vi "JSON RPC Engine.vi"(8 "error in (no error)":errorcluster, 10 "methods directory":path) -> (0 "error out":errorcluster)   [LabVIEW 2017, in "JSONRPC Server.lvclass"]
doc: "Use this as a starting point for the RPC Server processing loop in your application"
uses:
  JSONRPC Server.lvclass
  Request/Request.lvclass/Request.ctl
  Request/request.Read method.vi
  Request/request.Read params.vi
  params/params.To JSON Tree.vi
  Add Response (Method Not Found from Request).vi
  Add Response (Result from Request).vi
  Add Response (Server Error from Request).vi
  Add Response (Internal Error from Request).vi
  Method Loader/Method Loader.lvclass
  Request/Request.lvclass
  <vilib>/National Instruments/Variant JSON API/Variant JSON API.lvlib
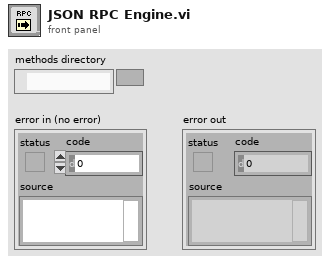
[diagram p1: front panel]
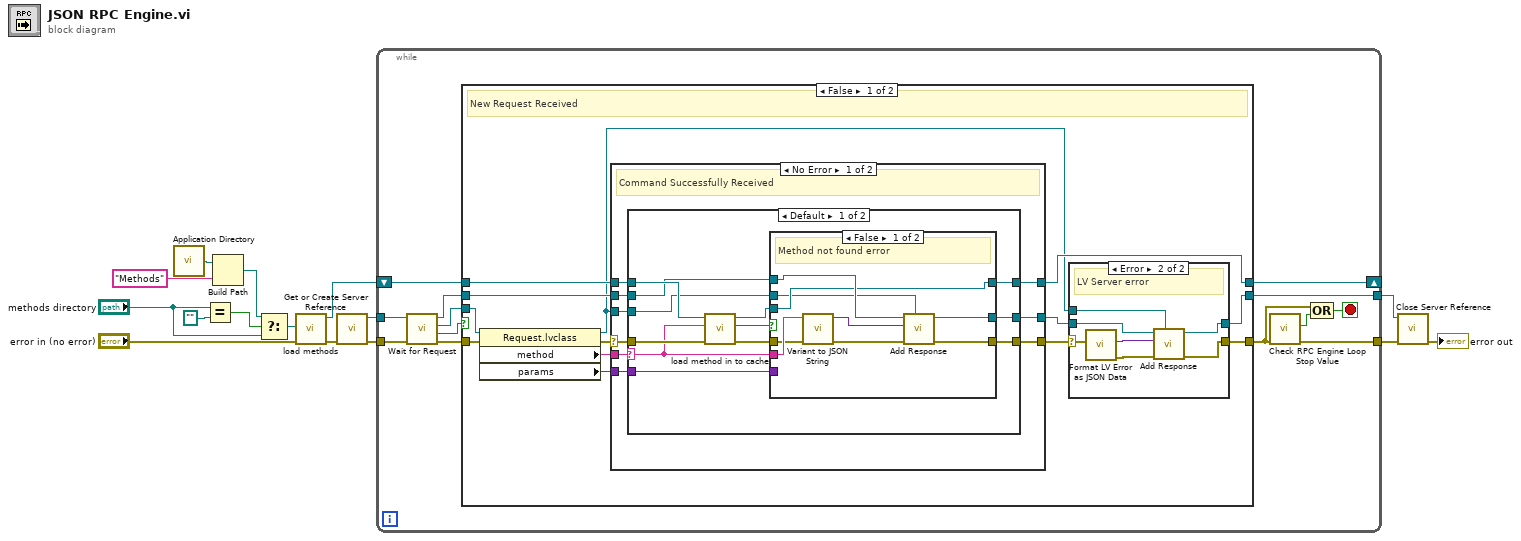
[diagram p0: block diagram]
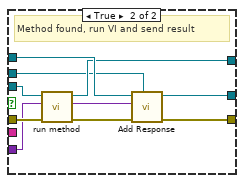
[diagram p3: hidden frame]
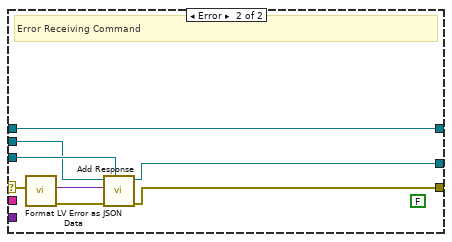
[diagram p5: hidden frame]
diagram:
  n1 = call <vilib>:"Application Directory.vi"() -> ("Application Directory"=w11:path)
  n2 = Equal?(x="methods directory", y=path "") -> (x = y?=w4:bool)
  n3 = Build Path(base path=w11, name or relative path="Methods") -> (appended path=w3:path)
  n4 = Select(t=w3, s=w4, f="methods directory") -> (s? t:f=w1:path)
  n5 = call "load methods.vi"("error in (no error)"="error in (no error)", "Folder Path"=w1) -> ("error out"=w9:errorcluster, "Method Manager out"=w8:refnum<class "Method Loader.lvclass">)  [unwired: 8 in]
  n6 = call "Get or Create Server Reference.vi"("error in (no error)"=w9) -> ("error out"=w14:errorcluster, "Server Out"=w15:refnum<class "JSONRPC Server.lvclass">)  [unwired: 9 in]
  n7 = while {
    tunnel: w15 -> [w28]
    tunnel: w14 -> [w24]
    tunnel: [w17] -> w12
    tunnel: [w22] -> w13
    shift-right: [w19] -> _
    shift-left: w8 -> [w20]
    stop <- w21 stop-if-true
    n8 = call "Wait for Request.vi"("error in (no error)"=w24, "Server in"=w28) -> ("error out"=w23:errorcluster, "timed out?"=w25:bool, "Request"=w26:refnum<class "Request.lvclass">, "Server out"=w27:refnum<class "JSONRPC Server.lvclass">)  [unwired: 6 in]
    n9 = case shown="False" w25 {
      tunnel: w27 -> [w36 w103]
      tunnel: w26 -> [w41 _]
      tunnel: w23 -> [w38 w104]
      tunnel: [w32 w104] -> w18
      tunnel: [w30 w103] -> w22
      tunnel: w20 -> [w35 w102]
      tunnel: [w34 w102] -> w19
      frame False {
        # "New Request Received"
        n10 = property class="Request.lvclass"(reference=w41, error in=w38) -> (reference out=w29:refnum<class "Request.lvclass">, error out=w37:errorcluster, "method"=w40:string, "params"=w39:variant)
        n11 = case shown="No Error" w37 {
          selector: w37 -> [w57 w96]
          tunnel: w40 -> [w59 _]
          tunnel: w39 -> [w51 _]
          tunnel: [w54 w98] -> w33
          tunnel: w36 -> [w56 w100]
          tunnel: [w53 w99] -> w31
          tunnel: w29 -> [w52 w101]
          tunnel: w35 -> [w58 w94]
          tunnel: [w55 w94] -> w34
          frame No Error {
            # "Command Successfully Received"
            n12 = case shown="Default" w59 {
              selector: w59 -> [w61 _]
              tunnel: w58 -> [w71 w93]
              tunnel: w57 -> [w67 w92]
              tunnel: w56 -> [w66 w91]
              tunnel: [w65 w93] -> w55
              tunnel: [w63 w92] -> w54
              tunnel: [w64 w91] -> w53
              tunnel: w52 -> [w62 _]
              tunnel: w51 -> [w60 _]
              frame Default {
                n13 = call "load method in to cache.vi"("error in (no error)"=w67, "method name"=w61, "Method Manager in"=w71) -> ("error out"=w68:errorcluster, "found?"=w70:bool, "Method Manager out"=w69:refnum<class "Method Loader.lvclass">)  [unwired: 6 in]
                n14 = case shown="False" w70 {
                  tunnel: w69 -> [w73 w90]
                  tunnel: w68 -> [w79 w89]
                  tunnel: w66 -> [w77 w88]
                  tunnel: [w73 w85] -> w65
                  tunnel: [w76 w83] -> w64
                  tunnel: [w74 w84] -> w63
                  tunnel: w62 -> [w72 w82]
                  tunnel: w61 -> [w80 _]
                  tunnel: w60 -> [_ w81]
                  frame False {
                    # "Method not found error"
                    n15 = call <vilib>:"Variant to JSON String.vi"("error in (no error)"=w79, "Variant in"=w80) -> ("error out"=w75:errorcluster, "Variant out"=w78:variant)  [unwired: 7 in, 1 out]
                    n16 = call-poly "Add Response.vi"("Request"=w72, "error in (no error)"=w75, "data"=w78, "Server in"=w77) -> ("error out"=w74:errorcluster, "Server out"=w76:refnum<class "JSONRPC Server.lvclass">)  [unwired: 5 in, 1 out]
                  }
                  frame True {
                    # "Method found, run VI and send result"
                    n17 = call "run method.vi"("error in (no error)"=w89, "JSON Value in"=w81, "Method Manager in"=w90) -> ("error out"=w87:errorcluster, "JSON Value out"=w86:variant, "Method Manager out"=w85:refnum<class "Method Loader.lvclass">)  [unwired: 6 in]
                    n18 = call-poly "Add Response.vi"("Request"=w82, "error in (no error)"=w87, "JSON Value in"=w86, "Server in"=w88) -> ("error out"=w84:errorcluster, "Server out"=w83:refnum<class "JSONRPC Server.lvclass">)  [unwired: 5 in, 1 out]
                  }
                }
              }
              frame "shutdown_rpc_server" {
              }
            }
          }
          frame Error {
            (unwired) FALSE
            # "Error Receiving Command"
            n19 = call "Format LV Error as JSON Data.vi"("error in"=w96) -> ("error out"=w97:errorcluster, "Error Value out"=w95:variant)  [unwired: 9 in]
            n20 = call-poly "Add Response.vi"("Request"=w101, "error in (no error)"=w97, "data"=w95, "Server in"=w100) -> ("error out"=w98:errorcluster, "Server out"=w99:refnum<class "JSONRPC Server.lvclass">)  [unwired: 5 in, 1 out]
          }
        }
        n21 = case shown="Error" w33 {
          selector: w33 -> [w43 w46]
          tunnel: [w43 w45] -> w32
          tunnel: w31 -> [w42 w49]
          tunnel: [w42 w48] -> w30
          tunnel: w29 -> [_ w44]
          frame No Error {
          }
          frame Error {
            # "LV Server error"
            n22 = call "Format LV Error as JSON Data.vi"("error in"=w46) -> ("error out"=w47:errorcluster, "Error Value out"=w50:variant)  [unwired: 9 in]
            n23 = call-poly "Add Response.vi"("Request"=w44, "error in (no error)"=w47, "data"=w50, "Server in"=w49) -> ("error out"=w45:errorcluster, "Server out"=w48:refnum<class "JSONRPC Server.lvclass">)  [unwired: 5 in, 1 out]
          }
        }
      }
      frame True {
        # "Timeout while waiting for new Requests"
      }
    }
    n24 = call "Check RPC Engine Loop Stop Value.vi"("error in (no error)"=w18) -> ("error out"=w17:errorcluster, "stopped?"=w16:bool)  [unwired: 9 in]
    n25 = Compound Arithmetic op=OR(w18, w16) -> (w21:bool)
  }
  n26 = call "Close Server Reference.vi"("error in (no error)"=w12, "Server in"=w13) -> ("error out"=→"error out":errorcluster)  [unwired: 9 in]
